vi "AlliGator Decay Graph Panel.vi"() -> ()   [LabVIEW 2021, in "AlliGator Decay Graph.lvlib"]
uses:
  AlliGator Decay Graph.lvlib
  AlliGator Decay Graph Ctrl Refnums.ctl
  Globals, Variables, Constants/AlliGator Refnums List.ctl
  Settings/AlliGator Settings List.ctl
  Graphs/XY Graph/XY Graph Event.ctl
  <vilib>/Utility/miscctls.llb/LVPoint32TypeDef.ctl
  Action Engine/AlliGator Q Element.ctl
  Action Engine/AlliGator Q Event.ctl
  Variant/Variant to Data/Variant to Boolean.vi
  Settings/AlliGator Settings+.lvlib
  Variant/Variant to Data/Variant to Data.lvlib
  Notebook/Notebook.lvlib
  Action Engine/AlliGator Action Engine.lvlib
  GUI/GUI.lvlib
  GUI/AlliGator GUI.lvlib
  Error/Error.lvlib
  Graphs/XY Graph/XY Graph Add-Ons.lvlib
  Python Plugins API/AlliGator Python Plugins.lvlib
  Decay Analysis/Decay Processing/AlliGator Decay Processing.lvlib
  Utilities/Utilities.lvlib
panel:
  out "Decay Integrated Intensity":dbl=46949635.0 caption="Bkgd-subtracted Intensity" format="%#_5g"
  out "Decay Background":dbl caption="Background" format="%#_5g"
  out "Decay Lifetime":dbl[unit] caption="Lifetime" format="%#_5g"
  in  "Decay Graph Active":bool=TRUE
  in  "Pin Button":bool=TRUE
  out "Decay Graph TipStrip":string caption="Lifetime Graph TipStrip"
  out "Decay Graph":cluster{"X Array":dbl[], "Y Array":dbl[]}[](graph)
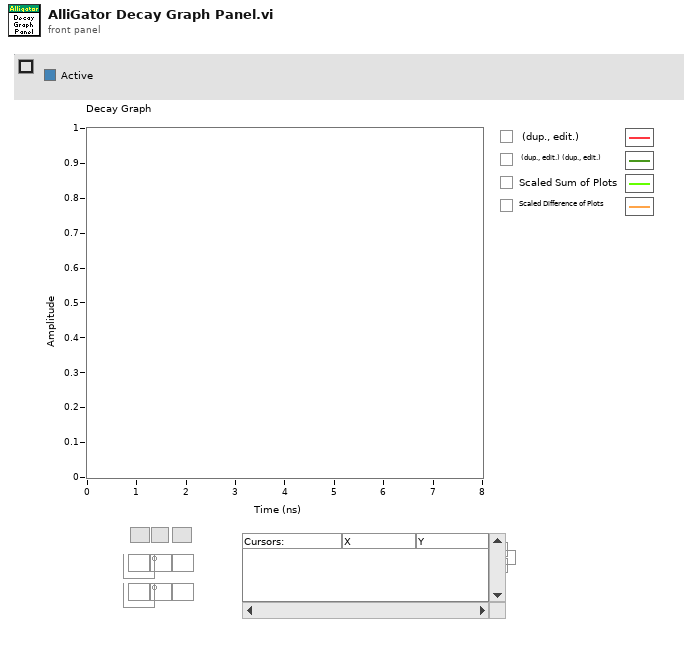
[diagram p1: front panel]
types:
  T1 = typedef "AlliGator GUI.lvlib/AlliGator Refnums List.ctl" = enum16{"---------- AlliGator Control Refnums ----------", "AlliGator Tab Control Refnum", "Dataset Ctrl Refnums", "Image Histogram Ctrl Refnums", "Intensity Time Trace Ctrl Refnums", "Decay Graph Ctrl Refnums", "Decay Statistics Graph Ctrl Refnums", "Phasor Graph Ctrl Refnums", "Phasor Ratio Graph Ctrl Refnums", "Phasor Plot Ctrl Refnums", "Lifetime & Other Parameters Ctrl Refnums", "Decay Fit Parameter Map Ctrl Refnums", "Parameter Map Ctrl Refnums", "Other AlliGator Ctrl Refnums", "---------- AlliGator Menu Refnums ----------", "AlliGator Menu", "---------- IO Device ID ----------", "Mouse ID", "Keyboard ID"}
  T2 = typedef "AlliGator Decay Graph.lvlib/AlliGator Decay Graph Ctrl Refnums.ctl" = cluster{"Decay Graph":refnum<vi>, "Decay Graph Active":refnum<vi>, "Decay Background":refnum<vi>, "Decay Integrated Intensity":refnum<vi>, "Decay Lifetime":refnum<vi>}
  T3 = cluster{"Event Registration Refnum":refnum<event-registration>, "Event Registration Refnum":refnum<event-registration>}
  T4 = typedef "AlliGator Settings+.lvlib/AlliGator Settings List.ctl" = enum16{"GUI:Visible Settings Tab", "GUI:Last Run Version", "Source Image:Use Image Histogram for Contrast", "Source Image:Low Count Pixels Rejection Options", "Source Image:High Count Pixels Rejection Options", "Source Image:Use Image Brightness", "Source Image:Blend Overlay with Image Background", "Source Image:Use Fixed ROI Diameter", "Source Image:ROI Diameter", "Source Image:ROI Center Color", "Source Image:Peak Threshold", "Source Image:Intensity Threshold", "Source Image:Image Binning Options", "Source Image:Image Smoothing Options", "Source Image:Image Histogram Active", "Source Image:Invert Binary Mask", "Source Image:Hot Pixel Removal", "Source Image:Overlay Analyzed ROI Center", "Source Image:Auto-Adjust Contrast", "Source Image:Histogram Lower Percentile", "Source Image:Histogram Upper Percentile", "Source Image:Lock ROI with Maps", "Source Image:Save Source Image", "Source Image:Scale Bar Options", "Source Image:Image Resolution (Pixel Size)", "Source Image:Flatfield Correction", "Source Image:Show Dead Left Columns Correction", "Source Image:Dead Left Columns Correction", "Source Image:Image Pre-Processing Operations Order", "Source Image:Overlay ROI Median", "Source Image:Median Overlay Color", "Data Information:Gate Width", "Data Information:Nanotime Gate Separation", "Data Information:Macrotime Gate Separation", "Data Information:Gate Step", "Data Information:# Gates", "Data Information:Gate Image Exposure", "Data Information:Gate Image Integration", "Data Information:Gates to Skip", "Data Information:Gates to Keep", "Data Information:Define Gates to", "Data Information:Channel Name", "Data Information:Available Channel Names", "Data Information:Channel Arithmetic", "Data Information:Background File Subtraction", "Data Information:Background File", "Data Information:Background Scaling Factor", "Data Information:Background Pile-up Correction", "Data Information:Background Pixel Well Capacity", "Data Information:Laser Period", "Data Information:SYNC Period", "Data Information:Pile-up Correction", "Data Information:Pixel Well Capacity", "Data Information:Dataset Scaling Factor", "Fluorescence Decay_Decay Pre-Processing:Reverse Gates", "Fluorescence Decay_Decay Pre-Processing:Verbose Decay Pre-Processing", "Fluorescence Decay_Decay Pre-Processing:Use Decay Pre-Processing", "Fluorescence Decay_Decay Pre-Processing:Background Subtraction", "Fluorescence Decay_Decay Pre-Processing:Background Definition Range", "Fluorescence Decay_Decay Pre-Processing:Baseline Subtraction Method", "Fluorescence Decay_Decay Pre-Processing:Decay Pre-Processing Operations Order", "Fluorescence Decay_Decay Pre-Processing:Smoothing Parameter", "Fluorescence Decay_Decay Pre-Processing:Shift Decay", "Fluorescence Decay_Decay Pre-Processing:Decay Shift Parameters", "Fluorescence Decay_Decay Pre-Processing:Fold Decay", "Fluorescence Decay_Decay Pre-Processing:# Folds", "Fluorescence Decay_Decay Pre-Processing:1-Normalize Decay", "Fluorescence Decay_Decay Pre-Processing:[0-1]-Normalize Decay", "Fluorescence Decay_Decay Pre-Processing:Smoothen Decay", "Fluorescence Decay_Decay Pre-Processing:Extrapolate Decay", "Fluorescence Decay_Decay Pre-Processing:Use Periodicity", "Fluorescence Decay_Decay Pre-Processing:Use Cursors", "Fluorescence Decay_Decay Pre-Processing:Tail Fraction", "Fluorescence Decay_Decay Pre-Processing:Head Fraction", "Fluorescence Decay_Decay Pre-Processing:Additional Points", "Fluorescence Decay_Decay Pre-Processing:Straighten Decay", "Fluorescence Decay_Decay Pre-Processing:Constant Background", "Fluorescence Decay_Decay Pre-Processing:Pixel-Normalize Decay", "Fluorescence Decay_Advanced Analysis:Extract IRF instead of Decay", "Fluorescence Decay_Advanced Analysis:IRF Extraction Options", "Fluorescence Decay_Advanced Analysis:IRF Optimization Options", "Fluorescence Decay_Advanced Analysis:Square Pulse Options", "Fluorescence Decay_Advanced Analysis:IRF Order", "Fluorescence Decay_Advanced Analysis:IRF Time Constants", "Fluorescence Decay_Advanced Analysis:Wavelet Analysis Options", "Fluorescence Decay_Advanced Analysis:Average Lifetime Options", "Fluorescence Decay_Fit Options:Fit Options", "Fluorescence Decay_Fit Options:Use Legacy Fitting Approach", "Fluorescence Decay_Fit Options:Use Data Information Laser Period", "Fluorescence Decay_Fit Parameters:Displayed Fit Parameters", "Fluorescence Decay_Fit Parameters:Fit Parameter Constraints", "Fluorescence Decay_Fit Parameters:Export Tabulated Results", "Fluorescence Decay_Fit Parameters:MLE Baseline Offset Type", "Fluorescence Decay_Fit Parameters:MLE Baseline Offset", "Fluorescence Decay_Fit Parameters:Guess Parameter Names", "Fluorescence Decay_Fit Parameters:Guess Parameter Values", "Fluorescence Decay_Fit Parameters:Guess Parameters Options", "Fluorescence Decay_Fit Parameters:Optimal Offset Selection Criterion", "Fluorescence Decay_Styles:Show Last Decay Only", "Fluorescence Decay_Styles:Decay Graph Color Array", "Fluorescence Decay:Decay Graph Active", "Fluorescence Decay Statistics:Min Peak Value", "Fluorescence Decay Statistics:Reject Low Decay Peak Pixels", "Fluorescence Decay Statistics:Reject High Decay Peak Pixels", "Fluorescence Decay Statistics:Max Peak Value", "Time Traces:Use File Timestamp", "Time Traces:Time Step", "Time Traces:Use Intensity Correction File", "Time Traces:Intensity Correction File", "Phasor Plot:Phasor Plot Smoothing Options", "Phasor Plot:Phasor Plot Size", "Phasor Plot:Phasor Plot Graphics Options", "Phasor Plot:Cumulative Phasor Plot", "Phasor Plot:Use Phasor Brightness", "Phasor Plot:Blend Overlay with Phasor Background", "Phasor Plot:Save Phasor Plot", "Phasor Plot:Show References", "Phasor Plot:Phasor Ratio Decay Range", "Phasor Plot:Exponential Fading", "Phasor Plot:Phasor Ratio Reference Colors", "Phasor Plot:Reference Radius", "Phasor Plot:Show Color Map Vertices", "Phasor Plot:Phasor Plot Active", "Phasor Plot:Phasor Ratio Color Map Type", "Phasor Plot:Phasor Ratio Color Map", "Phasor Plot:Phasor Ratio Display Range", "Phasor Plot:Selected Image ROI(s)", "Phasor Plot:All Image ROIs", "Phasor Plot:Selected Phasor Plot ROI(s)", "Phasor Plot:All Phasor Plot ROIs", "Phasor Plot:Phasor Ratio Color-Coded Quantity", "Phasor Plot:Store Phasor Harmonics", "Phasor Plot:Draw Reference Segment", "Phasor Plot:User-Defined Quantity", "Phasor Plot:Color Scale High Color", "Phasor Plot:Color Scale Low Color", "Phasor Plot:Intensity-weighted Phasor Plot", "Phasor Graph:Phasor Frequency", "Phasor Graph:Phasor Ratio Type", "Phasor Graph:Pixel-level Phasor Computation", "Phasor Graph:Save Phasor Graph", "Phasor Graph:Phasor Graph Active", "Phasor Graph:Phasor SDV Options", "Phasor Graph:Intensity-weighted Phasor Graph", "Phasor Graph:Define Shortest Lifetime as", "Phasor Calibration:Use Backup Calibration if needed", "Phasor Calibration:Backup Calibration Type", "Phasor Calibration:Calibration Type", "Phasor Calibration:Calibration Lifetime", "Phasor Calibration:Calibration Map Algorithm", "Single-Exponential Phasor Locus (SEPL):Gate Parameters", "Single-Exponential Phasor Locus (SEPL):User-defined Gate", "Single-Exponential Phasor Locus (SEPL):User-defined IRF", "Single-Exponential Phasor Locus (SEPL):Phasor Parameters", "Single-Exponential Phasor Locus (SEPL):Decay & IRF Parameters", "Single-Exponential Phasor Locus (SEPL):Display Parameters", "Lifetime Analysis:Decay Analysis Parameters", "Lifetime Analysis:Lifetime Map Active", "Plugins:Python Settings", "Miscellaneous:Verbose Mode", "Miscellaneous:Beep after Script", "Miscellaneous:Saved Image File Format", "Miscellaneous:Exported Gate Image Settings", "Miscellaneous:Include Loading in Timing", "Miscellaneous:Verbose Settings Mode", "Miscellaneous:Histogram Options", "Miscellaneous:Beep on Error", "Miscellaneous:# Logical Processors Used", "Miscellaneous:ROI Description Max Characters", "Miscellaneous:Verbose Error Mode", "Miscellaneous:Transparent Mask Color"}
  T5 = typedef "XY Graph Add-Ons.lvlib/XY Graph Event.ctl" = cluster{"Item Tag":string, "XY Graph Refnum":refnum<vi>, "Coords":T6, "Item Path":string}
  T6 = typedef "LVPoint32TypeDef.ctl" = cluster{"Horizontal":i32, "Vertical":i32}
  T7 = enum16{"0", "1", "2", "3", "4", "5", "6", "7", "8", "9", "A", "B", "C", "D", "E", "F", "G", "H", "I", "J", "K", "L", "M", "N", "O", "P", "Q", "R", "S", "T", "U", "V", "W", "X", "Y", "Z", "F1", "F2", "F3", "F4", "F5", "F6", "F7", "F8", "F9", "F10", "F11", "F12", "F13", "F14", "F15", "ADD", "BACK", "BACKSLASH", "CAPITAL", "COMMA", "DECIMAL", "DELETE", "DIVIDE", "DOWN", "END", "EQUALS", "ESCAPE", "GRAVE (`)", "HOME", "INSERT", "LBRACKET", "LCONTROL", "LEFT", "L ALT", "LSHIFT", "LWIN", "MINUS", "MULTIPLY", "NEXT", "NUMLOCK", "NUMPAD_0", "NUMPAD_1", "NUMPAD_2", "NUMPAD_3", "NUMPAD_4", "NUMPAD_5", "NUMPAD_6", "NUMPAD_7", "NUMPAD_8", "NUMPAD_9", "PAUSE", "PERIOD", "PRIOR (PG UP)", "RBRACKET", "RCONTROL", "RETURN", "RIGHT", "R ALT", "RSHIFT", "RWIN", "SCROLL", "SEMICOLON", "SLASH", "SPACE", "SUBTRACT", "TAB", "UP", "ENTER (num pad)", "' (quote)"}
  T8 = typedef "AlliGator Action Engine.lvlib/AlliGator Q Element.ctl" = cluster{"AlliGator Q Event":T9, "Data":variant}
  T9 = typedef "AlliGator Action Engine.lvlib/AlliGator Q Event.ctl" = enum16{"---- Files ----", "Files:Set Batch Export Files To Save", "Files:Set Dataset Loading & Pre-processing Options", "Files:Check #Frames in Dataset", "Files:Increment Frame Index", "Files:Open Mask Image", "Files:Open White Light Image", "Files:Open Single Dataset", "Files:New Folder of Folders Selected", "Files:Load File (all Types)_Scriptable", "Files:Move Flattened Series to Folders Series", "Files:Select Folder", "Files:Load FLI Dataset", "Files:Load Swiss SPAD 1 Dataset", "Files:Load Swiss SPAD 2 Dataset", "Files:Load .sdt FLI Dataset", "Files:Load .ptu FLI Dataset", "Files:Load .bin FLI Dataset", "Files:Load Single Gate Image Folder", "Files:Load I/m/phi Dataset (deprecated)", "Files:Load Single Image", "Files:Subtract Background File", "Files:Export FLI Dataset", "Files:Load HDF5 FLI Dataset", "Files:Set Destination File Path", "Files:Save Mask Image", "Files:Batch Conversion", "Files:New Folder Selected", "Files:Close FLI Dataset", "Files:Close FLI Dataset Series", "Files:Close White Light Image", "Files:Close Mask Image", "---- FLI Dataset ----", "FLI Dataset:Channel Arithmetic", "FLI Dataset:Export Average Lifetime Map as ASCII", "FLI Dataset:Export User-Defined Quantity Map as ASCII", "FLI Dataset:Python Function FLI Dataset Event", "FLI Dataset:ROI Analysis", "FLI Dataset:Tilted Logistic Square Gated IRF Characteristics Map", "FLI Dataset:Logistic Square Gated IRF Characteristics Map", "FLI Dataset:Square Gated IRF Characteristics Map", "FLI Dataset:Multi-ROI Single-Pixel Phasor Analysis", "FLI Dataset:Multi-ROI Single-Pixel NLSF Analysis", "FLI Dataset:All ROIs IRF Extraction", "FLI Dataset:All ROIs Decay Fit Non-Interactive (Fast + Individual IRF)", "FLI Dataset:All ROIs Phasor Analysis", "FLI Dataset:All ROIs Decay Fit", "FLI Dataset:Fluorescence Decay Statistics", "FLI Dataset:Update Decay Statistics Graph", "FLI Dataset:Get Decay from ROI", "FLI Dataset:All ROIs Average Lifetimes", "FLI Dataset:Save/Load Local IRFs", "FLI Dataset:Clear Local IRFs", "FLI Dataset:Phasor Calibration Maps (# Gates Series) Script", "FLI Dataset:Calibrated Phasor Map Series", "---- FLI Dataset Series ----", "FLI Dataset Series:Sum All Datasets in Series", "FLI Dataset Series:Add Dataset to Accumulated Dataset", "FLI Dataset Series:Display Accumulated Dataset", "FLI Dataset Series:Clear Dataset Series Sum", "FLI Dataset Series:Time-Series Analysis (NLSF)", "FLI Dataset Series:Time-Series Analysis (Phasor)", "---- Image ----", "Image:Update Image Profile Plots", "Image:Image Histogram Cursor Move", "Image:Image Histogram", "Image:Image Contrast", "Image:Set Image Histogram Cursor Move Flag", "Image:Clear Image Overlay", "Image:Use ROI as Search Area", "Image:Set ROI Diameter", "Image:Save Image Data as TIFF", "Image:Save Displayed Image with Overlay", "Image:Save Image Overlay Only", "Image:Save Image as Hot Pixel Mask", "Image:Change Source Image Color Palette", "Image:Copy Image to Clipboard", "Image:Source Image ROI Selection", "Image:Delete All ROIs", "Image:Delete All Unselected ROIs", "Image:Delete ROI", "Image:Merge All ROIs", "Image:Store ROI", "Image:Source Image ROI Storage", "Image:Export ROI Description to Notebook", "Image:Save ROI", "Image:Load ROI", "Image:Paste ROI Definition", "Image:Clear ROI", "Image:Identify ROIs in Mask Image", "Image:Create Complementary ROI", "Image:Create Contour ROI", "Image:Create ROI(s) from Pixels with Peak above Min_Scriptable", "Image:Create ROI(s) from Pixels with Intensity above Min_Scriptable", "Image:Compute ROI Statistics", "Image:Delete ROI(s) based on ROI Characteristics", "Image:Create ROI Grid", "Image:ROI to Individual Pixel ROIs", "Image:Python Function Source Image Event", "Image:Show Phasor Calibration Map ROI Centers", "Image:Convert ROI to Mask Image", "Image:Mouse Move", "Image:Mouse Up", "Image:Set Source Image Mouse Move Flag", "Image:Add Scale Bar Overlay", "Image:Delete Existing ROIs Option", "Image:Overlay ROI Median", "Image:Check Current ROI", "Image:Update True Pixel Value", "Image:Use ROI", "---- Decay ----", "Decay:Clear IRF/Reference Plot", "Decay:Add Decay to Graph", "Decay:Smoothen Plot", "Decay:Smoothen Plot Tail", "Decay:Average Selected Plots", "Decay:Extract IRF", "Decay:Optimal IRF Extraction", "Decay:Threshold IRF", "Decay:Fit to Model IRF", "Decay:Fit IRF to Square Gate", "Decay:Fit IRF to Logistic Square Gate", "Decay:Fit IRF to Tilted Logistic Square Gate", "Decay:Create Bounding Cursors Set", "Decay:Export Bounding Cursors Definition to Notebook", "Decay:Denoise Plot", "Decay:Compute Cumulative Function", "Decay:Use as Reference Decay", "Decay:Show Reference Decay/IRF", "Decay:Extrapolate Decay", "Decay:Create Head & Tail Bounding Cursors", "Decay:Store Cursor-defined Head & Tail Fractions", "Decay:Rebin Plot", "Decay:1-Normalize Decay", "Decay:[0-1]-Normalize Plot", "Decay:Straighten Decay", "Decay:Shift Decay", "Decay:Fold Decay", "Decay:Fit Decay", "Decay:Global Fit of Selected Decays", "Decay:Post Global Fit Script", "Decay:Add Global Fit Parameters to Graph", "Decay:Add Decay Parameter(s) to Plot (Graph)", "Decay:Export Decay to Phasor Graph", "Decay:Compute Average Lifetime", "Decay:Plot Convolution", "Decay:Graph Tip Strip Update", "---- Decay Statistics ----", "Decay Statistics:Tip Strip Update", "---- Intensity Time Trace ----", "Intensity Time Trace:Use File Timestamp", "Intensity Time Trace:Load Intensity Corrections File", "Intensity Time Trace:Clear Intensity Corrections File", "Intensity Time Trace:Tip Strip Update", "---- Phasor Plot ----", "Phasor Plot:Build Phasor Plot", "Phasor Plot:Change Phasor Plot Color Palette", "Phasor Plot:Adjust Phasor Plot Display Range", "Phasor Plot:Highlight Image ROI in Phasor Plot", "Phasor Plot:Save Phasor Plot Image with Overlay", "Phasor Plot:Export Complex Phasor Map", "Phasor Plot:Export Phasor Ratio Map", "Phasor Plot:Export Average Lifetime Map", "Phasor Plot:Compute Phase Lifetime Histogram", "Phasor Plot:Compute Phasor Ratio Histogram", "Phasor Plot:Compute Phase Lifetime vs Intensity Scatter Plot", "Phasor Plot:Weber 2-Component Decomposition", "Phasor Plot:Update Phasor Color Map Vertices", "Phasor Plot:Clear Phasor Overlay", "Phasor Plot:Use Segment Extremities as References", "Phasor Plot:Use UC/Segment Intersections as References", "Phasor Plot:Use UC/Principal Axis Intersections as References", "Phasor Plot:Use UC/Linear Fit Intersections as References", "Phasor Plot:Update Phasor Plot Reference", "Phasor Plot:Show Local Phasor Info in Phasor Plot", "Phasor Plot:Update Phasor Plot State", "Phasor Plot:Phasor Plot ROI Storage", "Phasor Plot:Phasor Plot ROI Selection", "Phasor Plot:Python Function Phasor Plot Event", "Phasor Plot:Overlay Phasor ROI, Ratio or Map in Source Image", "Phasor Plot:Compute Decay of Selected Phasors", "Phasor Plot:Phasor at Image Pixel", "Phasor Plot:Mouse Move", "Phasor Plot:Mouse Up", "Phasor Plot:Display Range Mouse Move", "Phasor Plot:Set Mouse Move Flag", "Phasor Plot:Update True Phasor Plot Value", "---- Phasor Graph ----", "Phasor Graph:Get Phasor Value", "Phasor Graph:Create New Phasor Plot Dialog", "Phasor Graph:Update Last Phasor Value", "Phasor Graph:Update Phasor (m, phi)", "Phasor Graph:Remove Single Phasor from Plot", "Phasor Graph:Add Single Phasor to Plot", "Phasor Graph:Remove Phasor Plot", "Phasor Graph:Remove Selected Phasor Plots", "Phasor Graph:Clear Phasor Data", "Phasor Graph:Clear Phasor Graph", "Phasor Graph:Cursor Move", "Phasor Graph:Draw Cursor Connecting Line", "Phasor Graph:Clear Cursor Connecting Line", "Phasor Graph:Find UC Intersection", "Phasor Graph:Use UC/Cursor-Defined Line Intersections", "Phasor Graph:Use Selected Plots Fitted Line/UC Intersections", "Phasor Graph:Use Selected Plots Principal Axis/UC Intersections", "Phasor Graph:Show Single Phasor", "Phasor Graph:Save Single Phasor Plot", "Phasor Graph:Save All Phasor Plots", "Phasor Graph:Load Phasor Plot(s)", "Phasor Graph:Phasor Multiplication", "Phasor Graph:Compute Average Phasor", "Phasor Graph:Compute Multiple Average Phasors (Selected Plots)", "Phasor Graph:Export Single Phasor Plot Phase Lifetimes", "Phasor Graph:Parameter 2 vs Parameter 1 Scatter Plot", "Phasor Graph:Use Cursor n Location", "Phasor Graph:Set Reference n to Current Phase Lifetime Value", "Phasor Graph:Set Reference n to Lifetime Value", "Phasor Graph:Set Cursor n Location", "Phasor Graph:Save Phasor Graph Image", "Phasor Graph:Update SEPL Plot", "Phasor Graph:Export Single Phasor Plot Data", "Phasor Graph:Export Selected Phasor Plots Data", "Phasor Graph:Python Function Phasor Graph Event", "Phasor Graph:Tip Strip Update", "---- Calibration ----", "Calibration:Set Calibration Type", "Calibration:Load/Save Phasor Calibration", "Calibration:Load/Save Phasor Calibration Series", "Calibration:Load/Save Phasor Calibration Map", "Calibration:Use as Calibration", "Calibration:Compute Optimal Calibration from Phasor References", "Calibration:Clear Phasor Calibration", "Calibration:Single Phasor Calibration Information", "Calibration:Use as Calibration Series", "Calibration:Use as Calibration Map", "Calibration:Clear Calibration Series", "Calibration:Phasor Calibration Series Information", "Calibration:Clear Calibration Map", "Calibration:Phasor Calibration Map Information", "Calibration:Apply Phasor Calibration", "Calibration:Update Single Plot Calibration", "Calibration:Update Multiple Plots Calibration", "Calibration:Clear Single Plot Calibration", "Calibration:Clear All Plots Calibrations", "Calibration:Clear Plot(s) Calibration(s)?", "---- Phasor Ratio ----", "Phasor Ratio:Clear Reference n", "Phasor Ratio:Toggle Selected Plot(s)  Lock to Reference 1", "Phasor Ratio:Use as Reference n", "Phasor Ratio:Send Reference n to Notebook", "Phasor Ratio:Toggle Selected Plot(s)  Lock to Reference 2", "Phasor Ratio:Compute Phasor Ratio at Mouse Location", "Phasor Ratio:Compute Phasor Plot's Average Phasor Ratio", "Phasor Ratio:Compute Time-Series Phasor Ratios", "Phasor Ratio:Fit Line to Phasor Ratio Plot", "Phasor Ratio:Save References", "Phasor Ratio:Load References", "Phasor Ratio:Update Phasor Reference 1", "Phasor Ratio:Update Phasor Reference 2", "Phasor Ratio:Move Cursor n to Reference n", "Phasor Ratio:Use as Phasor Reference 1 Lifetime", "Phasor Ratio:Use as Phasor Reference 2 Lifetime", "Phasor Ratio:Export Phasor Ratio Map as ASCII", "Phasor Ratio:Tip Strip Update", "---- Lifetime & Other Parameters Graph ----", "Lifetime:Compute Sliced Mean, SDV and CV Plots", "Lifetime:Plot Decay Shifts", "Lifetime:Plot Histogram", "---- Decay Fit Parameter Map ----", "Decay Fit Parameter Map:Export ROI NLSF Data as ASCII", "Decay Fit Parameter Map:Set Decay Fit Parameter Map Selection", "Decay Fit Parameter Map:Build Decay Fit Parameter Map", "Decay Fit Parameter Map:Change Decay Fit Parameter Map Color Palette", "Decay Fit Parameter Map:Export Decay Fit Parameter Map Data as ASCII", "Decay Fit Parameter Map:Export All Decay Fit Parameter Maps Data as ASCII", "Decay Fit Parameter Map:Selected Parameter Scatterplot", "Decay Fit Parameter Map:Parameter 2 vs Parameter 1 Scatterplot", "Decay Fit Parameter Map:Save Decay Fit Parameter Map Image", "Decay Fit Parameter Map:Save-Load IRFs & Fit Data", "Decay Fit Parameter Map:Update Local Decay Plots", "Decay Fit Parameter Map:Python Function Decay Fit Parameters Map Event", "Decay Fit Parameter Map:Overlay Decay Fit Parameter Map in Source Image", "Decay Fit Parameter Map:Selected Parameter vs Intensity Scatterplot", "Decay Fit Parameter Map:Mouse Up", "Decay Fit Parameter Map:Mouse Move", "Decay Fit Parameter Map:Display Range Mouse Move", "Decay Fit Parameter Map:Change Map Resolution", "Decay Fit Parameter Map:Variance Significance Maps", "Decay Fit Parameter Map:Fit Result Constraints Window", "Decay Fit Parameter Map:Use ROI", "---- Parameter Map ----", "Parameter Map:Export ROI Parameters Data as ASCII", "Parameter Map:Add Parameter Map Set", "Parameter Map:Delete Parameter Map Set", "Parameter Map:Update Parameter List", "Parameter Map:Build Parameter Map", "Parameter Map:Change Parameter Map Color Palette", "Parameter Map:Export Parameter Map Data as ASCII", "Parameter Map:Export All Parameter Maps Data as ASCII", "Parameter Map:Selected Parameter Scatterplot", "Parameter Map:Parameter 2 vs Parameter 1 Scatterplot", "Parameter Map:Selected Parameter vs Intensity Scatterplot", "Parameter Map:Save Parameter Map Image", "Parameter Map:Save-Load IRFs & Parameter Maps (TODO)", "Parameter Map:Set Parameter Map Selection", "Parameter Map:Python Function Parameter Map Event", "Parameter Map:Overlay Parameter Map in Source Image", "Parameter Map:Update Local Decay Plots", "Parameter Map:Mouse Up", "Parameter Map:Mouse Move", "Parameter Map:Display Range Mouse Move", "Parameter Map:Use ROI", "---- Generic Graph ----", "Generic Graph:Generic XY Graph Event", "Generic Graph:Python Function XY Graph Event", "Generic Graph:New Plot", "Generic Graph:Save Plot", "Generic Graph:XY Plot Histogram", "Generic Graph:Set XY Graph Plot Name", "Generic Graph:Set Last Cursor Style", "Generic Graph:Tip Strip Update", "---- GUI ----", "GUI:Start Script", "GUI:Type of Displayed Image Changed", "GUI:Gate Image Slide Changed", "GUI:Show Busy Icon", "GUI:Show Busy Icon & Abort Button", "GUI:Hide Busy Icon", "GUI:Hide Busy Icon & Abort Button", "GUI:Abort", "GUI:End Script", "GUI:Start Timing", "GUI:End Timing", "GUI:Set State Indicator", "GUI:Send Parameters JSON Strings to Clipboard", "GUI:Set Gate Step", "GUI:Idle", "GUI:Initialization", "GUI:Quit", "GUI:Increment Dataset Index", "GUI:Set Dataset Index to -1", "GUI:Time Series Slider Moved", "GUI:Time Series Slider Changed", "GUI:Toggle Playback or Loop", "GUI:Playback Script", "GUI:Set Phasor Frequency", "GUI:Open Window", "GUI:Start Test Script", "GUI:End Test Script", "GUI:Set Verbose Mode", "GUI:Set Verbose Settings Mode", "GUI:Initialize Python Session", "DEBUG"}
  T10 = enum16{"0", "1", "2", "3", "4", "5", "6", "7", "8", "9", "A", "B", "C", "D", "E", "F", "G", "H", "I", "J", "K", "L", "M", "N", "O", "P", "Q", "R", "S", "T", "U", "V", "W", "X", "Y", "Z", "F1", "F2", "F3", "F4", "F5", "F6", "F7", "F8", "F9", "F10", "F11", "F12", "F13", "F14", "F15", "ADD", "BACK", "BACKSLASH", "CAPITAL", "COMMA", "DECIMAL", "DELETE", "DIVIDE", "DOWN", "END", "EQUALS", "ESCAPE", "GRAVE (`)", "HOME", "INSERT", "LBRACKET", "LCONTROL", "LEFT", "L ALT", "LSHIFT", "LWIN", "MINUS", "MULTIPLY", "NEXT", "NUMLOCK", "NUMPAD_0", "NUMPAD_1", "NUMPAD_2", "NUMPAD_3", "NUMPAD_4", "NUMPAD_5", "NUMPAD_6", "NUMPAD_7", "NUMPAD_8", "NUMPAD_9", "PAUSE", "PERIOD", "PRIOR (PG UP)", "RBRACKET", "RCONTROL", "RETURN", "RIGHT", "R ALT", "RSHIFT", "RWIN", "SCROLL", "SEMICOLON", "SLASH", "SPACE", "SUBTRACT", "TAB", "UP", "ENTER (num pad)", "' (quote)"}[]
  T11 = typedef "XY Graph Add-Ons.lvlib/XY Graph Refnum.ctl" = refnum<vi>
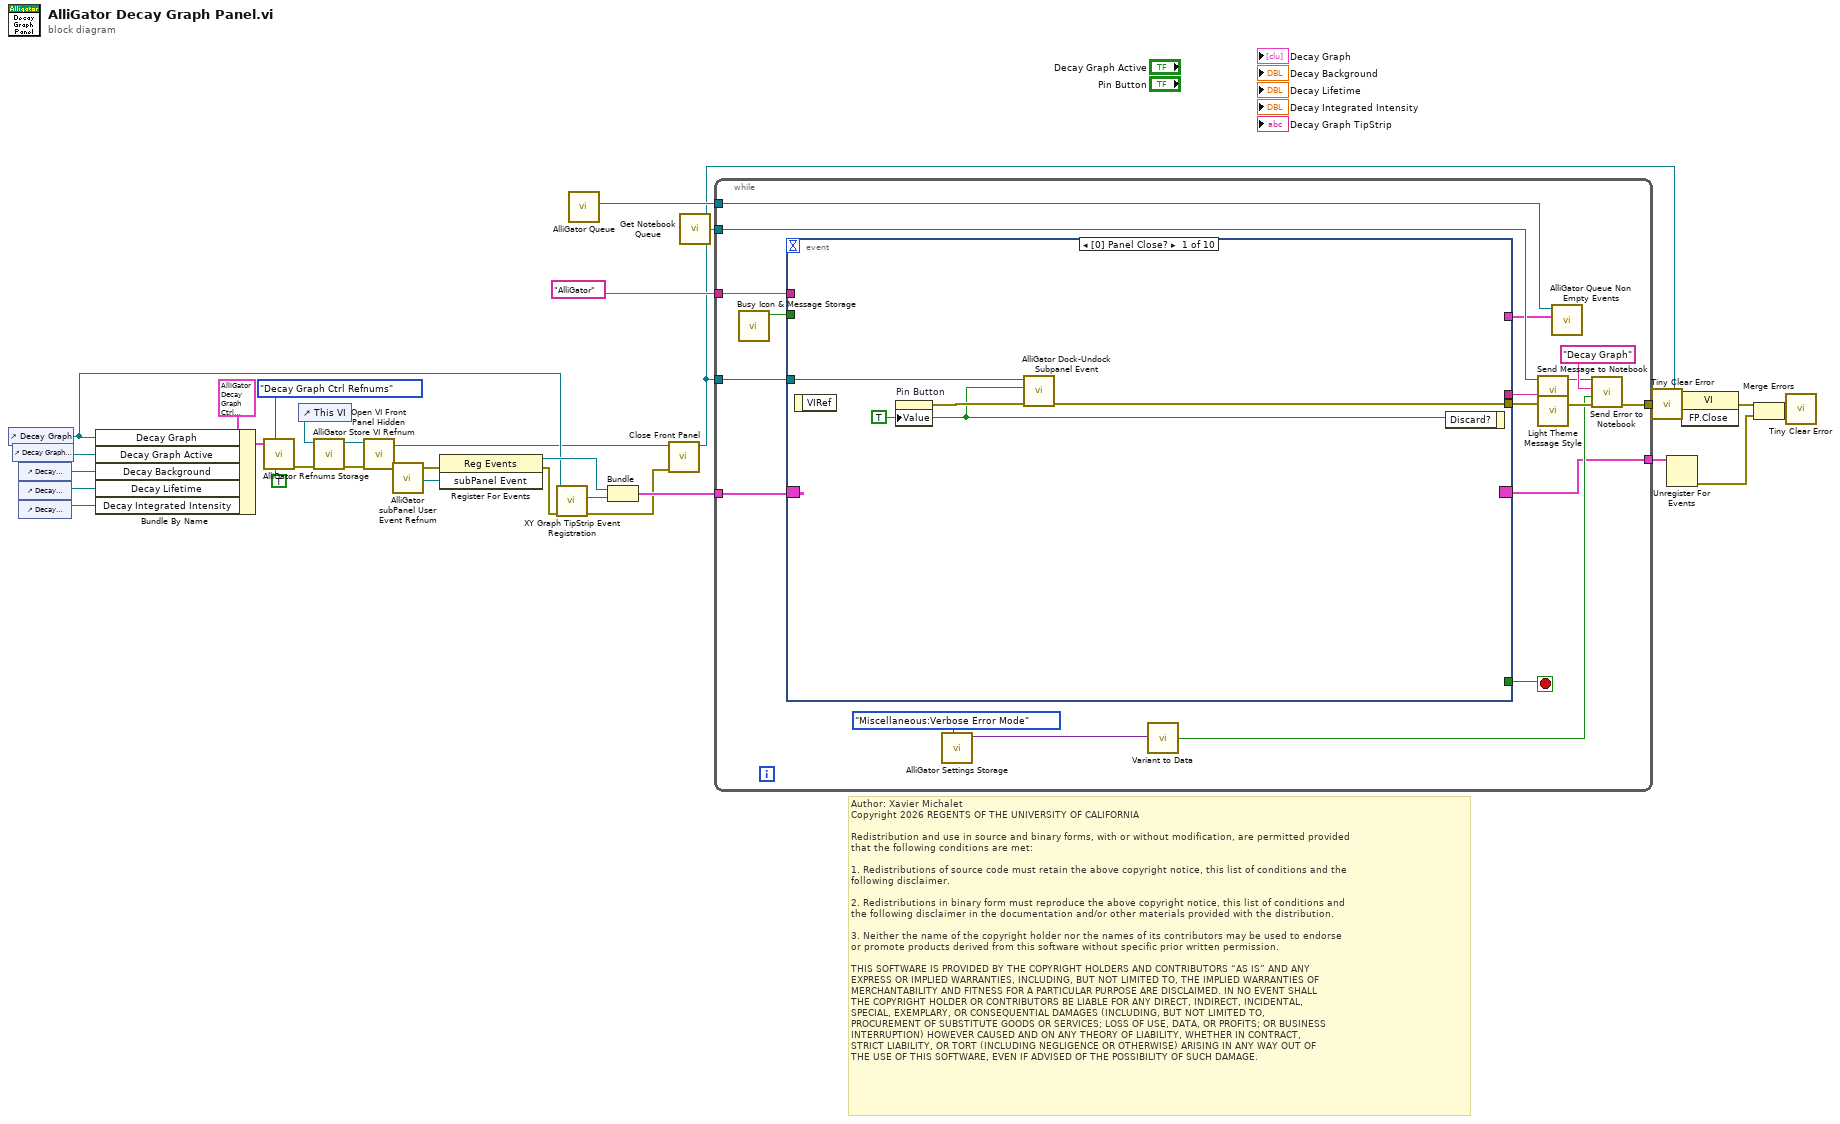
[diagram p0: block diagram]
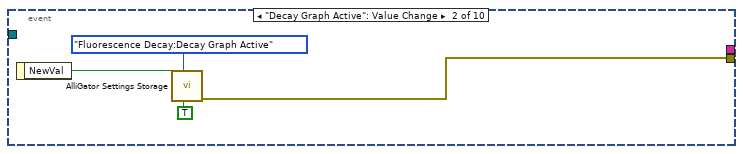
[diagram p2: hidden frame]
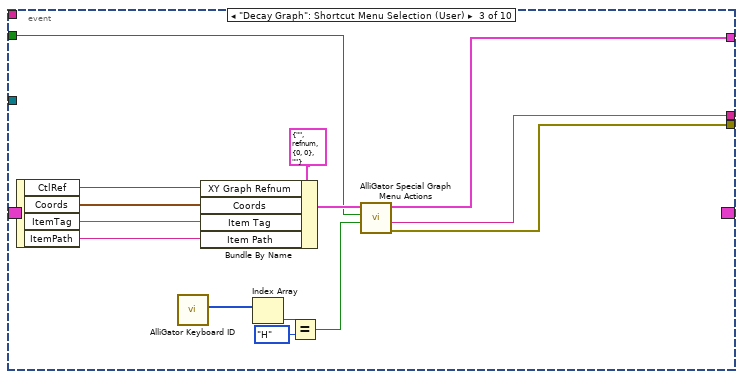
[diagram p3: hidden frame]
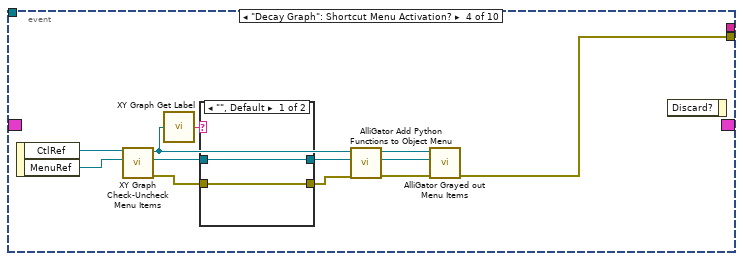
[diagram p4: hidden frame]
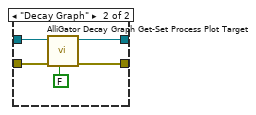
[diagram p5: hidden frame]
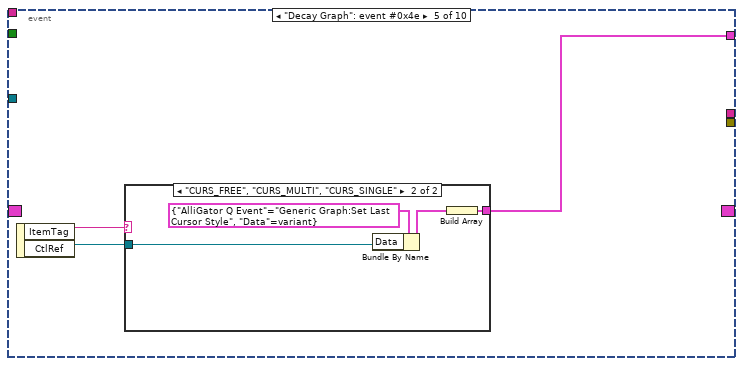
[diagram p6: hidden frame]
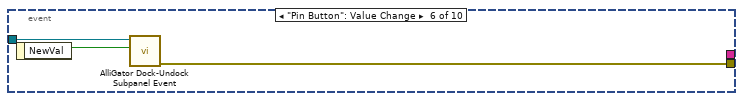
[diagram p8: hidden frame]
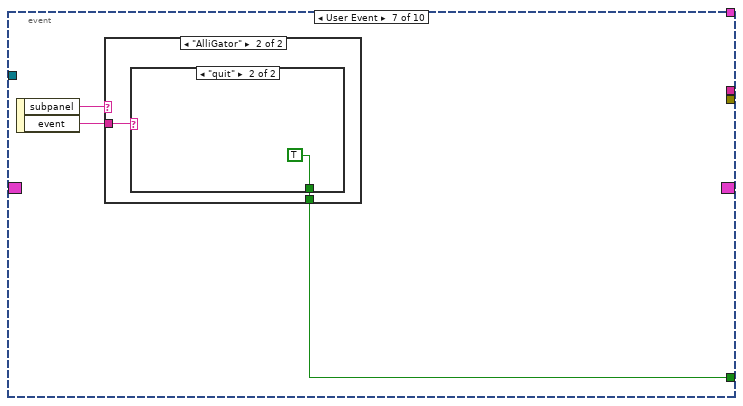
[diagram p9: hidden frame]
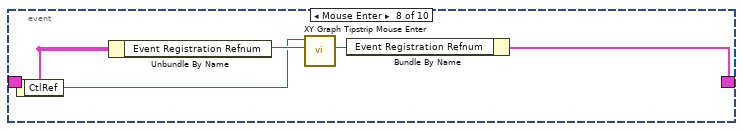
[diagram p12: hidden frame]
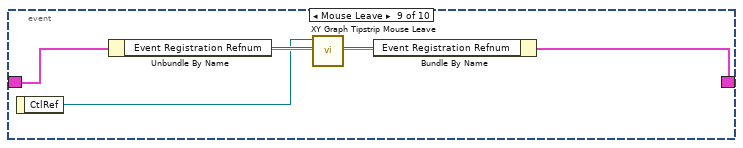
[diagram p13: hidden frame]
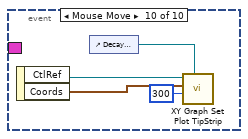
[diagram p14: hidden frame]
diagram:
  # "Author: Xavier Michalet\nCopyright 2026 REGENTS OF THE UNIVERSITY OF CALIFORNIA\n\nRedistribution and use in source and binary forms, with or without modification, are permitted provided\nthat the following conditions are met:\n\n1. Redistributions of source code must retain the above copyright notice, this list of conditions and the\nfollowing disclaimer.\n\n2. Redistributions in binary form must reproduce the above copyright notice, this list of conditions and\nthe following disclaimer in the documentation and/or other materials provided with the distribution.\n\n3. Neither the name of the copyright holder nor the names of its contributors may be used to endorse \nor promote products derived from this software without specific prior written permission.\n\nTHIS SOFTWARE IS PROVIDED BY THE COPYRIGHT HOLDERS AND CONTRIBUTORS “AS IS” AND ANY \nEXPRESS OR IMPLIED WARRANTIES, INCLUDING, BUT NOT LIMITED TO, THE IMPLIED WARRANTIES OF\nMERCHANTABILITY AND FITNESS FOR A PARTICULAR PURPOSE ARE DISCLAIMED. IN NO EVENT SHALL\nTHE COPYRIGHT HOLDER OR CONTRIBUTORS BE LIABLE FOR ANY DIRECT, INDIRECT, INCIDENTAL, \nSPECIAL, EXEMPLARY, OR CONSEQUENTIAL DAMAGES (INCLUDING, BUT NOT LIMITED TO, \nPROCUREMENT OF SUBSTITUTE GOODS OR SERVICES; LOSS OF USE, DATA, OR PROFITS; OR BUSINESS\nINTERRUPTION) HOWEVER CAUSED AND ON ANY THEORY OF LIABILITY, WHETHER IN CONTRACT, \nSTRICT LIABILITY, OR TORT (INCLUDING NEGLIGENCE OR OTHERWISE) ARISING IN ANY WAY OUT OF\nTHE USE OF THIS SOFTWARE, EVEN IF ADVISED OF THE POSSIBILITY OF SUCH DAMAGE."
  n1 = control-ref of="Decay Graph"() -> (w18:refnum<vi>)
  n2 = control-ref of="Decay Graph Active"() -> (w19:refnum<vi>)
  n3 = control-ref of="Decay Background"() -> (w7:refnum<vi>)
  n4 = control-ref of="Decay Lifetime"() -> (w6:refnum<vi>)
  n5 = control-ref of="Decay Integrated Intensity"() -> (w5:refnum<vi>)
  n6 = Bundle By Name(cluster=T2 {"Decay Graph"=refnum, "Decay Graph Active"=refnum, "Decay Background"=refnum, "Decay Integrated Intensity"=refnum, "Decay Lifetime"=refnum} ("Decay Graph Ctrl Refnums"), "Decay Graph"=w18, "Decay Graph Active"=w19, "Decay Background"=w7, "Decay Lifetime"=w6, "Decay Integrated Intensity"=w5) -> (w20:T2)
  n7 = call "AlliGator Refnums Storage.vi"("Get(F)/Set"=TRUE, "AlliGator Refnum List"=AlliGator_Refnums_List."Decay Graph Ctrl Refnums", "Data in"=w20) -> ("Error Out"=w2:errorcluster)  [unwired: 7 in, 1 out]
  n8 = control-ref of="This VI"() -> (w4:refnum<vi>)
  n9 = call "AlliGator Store VI Refnum.vi"("error in (no error)"=w2, "VI Refnum"=w4) -> ("error out"=w1:errorcluster, "VI Refnum (dup)"=w3:refnum<vi>)  [unwired: 7 in, 1 out]
  n10 = call "Open VI Front Panel Hidden.vi"("error in"=w1, "VI in"=w3) -> ("error out"=w12:errorcluster, "VI out"=w11:refnum<vi>)  [unwired: 8 in]
  n11 = call "AlliGator subPanel User Event Refnum.vi"() -> ("subPanel Event"=w28:refnum<user-event>)  [unwired: 9 in]
  n12 = register-events(error in=w12, w28) -> (reference out=w27:refnum<event-registration>, error out=w9:errorcluster)  [unwired: 1 in]
  n13 = call "XY Graph TipStrip Event Registration.vi"("error in (no error)"=w9, "XY Graph Refnum"=w18) -> ("error out"=w8:errorcluster, "Event Registration Refnum"=w16:refnum<event-registration>)  [unwired: 7 in, 1 out]
  n14 = call "AlliGator Queue.vi"() -> ("AlliGator Q"=w30:refnum<queue>)  [unwired: 8 in, 1 out]
  n15 = Bundle("Event Registration Refnum"=w27, "Event Registration Refnum"=w16) -> (w17:T3)  [unwired: 1 in]
  n16 = call "Close Front Panel.vi"("error in (no error)"=w8, "VI in"=w11) -> ("VI out"=w10:refnum<vi>)  [unwired: 8 in, 1 out]
  n17 = call "Get Notebook Queue.vi"() -> ("Notebook Queue"=w31:refnum<queue>)  [unwired: 9 in]
  n18 = while {
    tunnel: w31 -> [w42]
    tunnel: w30 -> [w39]
    tunnel: "AlliGator" ("Sender") -> [w37]
    tunnel: w10 -> [w35]
    tunnel: w17 -> [w34]
    tunnel: [w33] -> w26
    tunnel: [w32] -> w25
    stop <- w49 stop-if-true
    n19 = call "Busy Icon & Message Storage.vi"() -> ("Busy Icon Status (F = busy)"=w36:bool)  [unwired: 9 in, 2 out]
    n20 = event shown="[0] Panel Close?" {
      selector: w34 -> [_ _ _ _ _ _ _ w109 w114 _]
      dyn-events: [_ _ _ _ _ _ _ w107 w112 _] -> w33
      timeout: _ -> [_ _ _ _ _ _ _ _ _ _]
      tunnel: [w52 w54 w58 w72 _ w98 _ _ _ _] -> w43
      tunnel: [_ _ _ _ _ _ w101 _ _ _] -> w49
      tunnel: [_ _ w59 _ _ _ _ _ _ _] -> w40
      tunnel: [_ _ w60 _ w91 _ _ _ _ _] -> w38
      tunnel: w36 -> [_ _ w65 _ _ _ _ _ _ _]
      tunnel: w37 -> [_ _ _ _ _ _ _ _ _ _]
      tunnel: w35 -> [w51 _ _ _ _ w100 _ _ _ _]
      event Panel Close? {
        w50 = TRUE ("Pin Button")
        n21 = event-data() -> ()  [unwired: 1 in, 1 out]
        n22 = property on="Pin Button" class="Bool (strict)"("Value"=w50) -> (error out=w53:errorcluster)  [unwired: 2 in, 1 out]
        n23 = call "AlliGator Dock-Undock Subpanel Event.vi"("Error In"=w53, "Dock?"=w50, "VI in"=w51) -> ("Error Out"=w52:errorcluster)  [unwired: 8 in]
        n24 = event-data("Discard?"=w50) -> ()  [unwired: 1 in, 1 out]
      }
      event "Decay Graph Active": Value Change {
        n25 = event-data() -> ("NewVal"=w56:bool)  [unwired: 1 in]
        n26 = call "AlliGator Settings Storage.vi"("Get(F)/Set"=TRUE, "AlliGator Settings List"=AlliGator_Settings_List."Fluorescence Decay:Decay Graph Active", "Variant Data in"=w56) -> ("Error Out"=w54:errorcluster)  [unwired: 7 in, 1 out]
      }
      event "Decay Graph": Shortcut Menu Selection (User) {
        n27 = event-data() -> ("CtlRef"=w61:refnum<vi>, "Coords"=w64:T6, "ItemTag"=w62:string, "ItemPath"=w63:string)  [unwired: 1 in]
        n28 = call "AlliGator Keyboard ID.vi"() -> ("keys pressed"=w71:T10)  [unwired: 9 in, 2 out]
        n29 = Bundle By Name(cluster=T5 {"Item Tag"="", "XY Graph Refnum"=refnum, "Coords"={"Horizontal"=0, "Vertical"=0}, "Item Path"=""} ("XY Graph Event"), "XY Graph Refnum"=w61, "Coords"=w64, "Item Tag"=w62, "Item Path"=w63) -> (w69:T5)
        n30 = Index Array(array=w71) -> (element=w66:T7)  [unwired: 1 in]
        n31 = Equal?(x=w66, y=T7."H" ("element")) -> (x = y?=w70:bool)
        n32 = call "AlliGator Special Graph Menu Actions.vi"("Help?"=w70, "Animated Busy Icon"=w65, "XY Graph Event"=w69) -> ("Error Out"=w58:errorcluster, "Message"=w59:string, "AlliGator Actions"=w60:T8[])  [unwired: 6 in]
      }
      event "Decay Graph": Shortcut Menu Activation? {
        n33 = event-data() -> ("CtlRef"=w74:refnum<vi>, "MenuRef"=w73:refnum<k9>)  [unwired: 1 in]
        n34 = call "XY Graph Check-Uncheck Menu Items.vi"("Menu in"=w73, "XY Graph Refnum"=w74) -> ("Error Out (dup)"=w83:errorcluster, "Menu out"=w78:refnum<k9>, "XY Graph Refnum dup"=w76:T11)  [unwired: 6 in, 1 out]
        n35 = call "XY Graph Get Label.vi"("XYGraph"=w76) -> ("Graph Label"=w75:string)  [unwired: 8 in]
        n36 = case shown="\"\", Default" w75 {
          tunnel: w83 -> [w84 w90]
          tunnel: [w84 w89] -> w79
          tunnel: w78 -> [w85 w88]
          tunnel: [w85 w87] -> w77
          frame "", Default {
          }
          frame "Decay Graph" {
            n37 = call "AlliGator Decay Graph Get-Set Process Plot Target.vi"("Get (F)/Set"=FALSE, "Error In"=w90, "Menu"=w88) -> ("Error Out (dup)"=w89:errorcluster, "Menu"=w87:refnum<k9>)  [unwired: 6 in, 1 out]
          }
        }
        n38 = call "AlliGator Add Python Functions to Object Menu.vi"("error in (no error)"=w79, "Menu in"=w77, "Object Refnum"=w76) -> ("error out"=w82:errorcluster, "Menu out"=w81:refnum<k9>, "Object Refnum dup"=w80:refnum<vi>)  [unwired: 6 in]
        n39 = call "AlliGator Grayed out Menu Items.vi"("error in (no error)"=w82, "Menu in"=w81, "Object Refnum"=w80) -> ("error out"=w72:errorcluster)  [unwired: 7 in, 1 out]
        n40 = event-data() -> ()  [unwired: 2 in, 1 out]
      }
      event "Decay Graph": event #0x4e {
        n41 = event-data() -> ("ItemTag"=w92:string, "CtlRef"=w93:refnum<vi>)  [unwired: 1 in]
        n42 = case shown="\"CURS_FREE\", \"CURS_MULTI\", \"CURS_SINGLE\"" w92 {
          tunnel: w93 -> [_ w94]
          tunnel: [_ w96] -> w91
          frame "", Default {
          }
          frame "CURS_FREE", "CURS_MULTI", "CURS_SINGLE" {
            n43 = Bundle By Name(cluster=T8 {"AlliGator Q Event"=enum."Generic Graph:Set Last Cursor Style", "Data"=variant} ("AlliGator Actions"), "Data"=w94) -> (w95:T8)
            n44 = Build Array(w95) -> (w96:T8[])
          }
        }
      }
      event "Pin Button": Value Change {
        n45 = event-data() -> ("NewVal"=w99:bool)  [unwired: 1 in]
        n46 = call "AlliGator Dock-Undock Subpanel Event.vi"("Dock?"=w99, "VI in"=w100) -> ("Error Out"=w98:errorcluster)  [unwired: 9 in]
      }
      event User Event {
        n47 = event-data() -> ("subpanel"=w103:string, "event"=w102:string)  [unwired: 1 in]
        n48 = case shown="\"AlliGator\"" w103 {
          tunnel: w102 -> [_ w105]
          tunnel: [_ w104] -> w101
          frame "False", Default {
          }
          frame "AlliGator" {
            n49 = case shown="\"quit\"" w105 {
              tunnel: [_ TRUE] -> w104
              frame "False", Default {
              }
              frame "quit" {
              }
            }
          }
        }
      }
      event Mouse Enter {
        n50 = event-data() -> ("CtlRef"=w108:refnum<vi>)  [unwired: 1 in]
        n51 = Unbundle By Name(w109) -> ("Event Registration Refnum"=w111:refnum<event-registration>)
        n52 = call "XY Graph Tipstrip Mouse Enter.vi"("Event Registration Refnum"=w111, "XY Graph Refnum"=w108) -> ("Event Registration Refnum"=w110:refnum<event-registration>)  [unwired: 8 in, 1 out]
        n53 = Bundle By Name(cluster=w109, "Event Registration Refnum"=w110) -> (w107:T3)
      }
      event Mouse Leave {
        n54 = event-data() -> ("CtlRef"=w113:refnum<vi>)  [unwired: 1 in]
        n55 = Unbundle By Name(w114) -> ("Event Registration Refnum"=w115:refnum<event-registration>)
        n56 = call "XY Graph Tipstrip Mouse Leave.vi"("Event Registration Refnum"=w115, "XY Graph Refnum"=w113) -> ("Event Registration Refnum"=w116:refnum<event-registration>)  [unwired: 8 in, 1 out]
        n57 = Bundle By Name(cluster=w114, "Event Registration Refnum"=w116) -> (w112:T3)
      }
      event Mouse Move {
        n58 = event-data() -> ("CtlRef"=w119:refnum<vi>, "Coords"=w118:T6)  [unwired: 1 in]
        n59 = control-ref of="Decay Graph TipStrip"() -> (w117:refnum<vi>)
        n60 = call "XY Graph Set Plot TipStrip.vi"("TipStrip Refnum"=w117, "Max Length (200)"=300, "Coords"=w118, "XY Graph Refnum"=w119) -> ()  [unwired: 5 in, 3 out]
      }
    }
    n61 = call "AlliGator Settings Storage.vi"("AlliGator Settings List"=AlliGator_Settings_List."Miscellaneous:Verbose Error Mode") -> ("Variant Data out"=w48:variant)  [unwired: 9 in, 1 out]
    n62 = call-poly "Variant to Data.vi"("Variant"=w48) -> ("Value"=w41:bool)  [unwired: 8 in]
    n63 = call "Send Message to Notebook.vi"("Error In"=w43, "Text"=w40, "Notebook Queue"=w42) -> ("Error Out"=w45:errorcluster, "Notebook Queue"=w44:refnum<queue>)  [unwired: 5 in]
    n64 = call "Light Theme Message Style.vi"() -> ()  [unwired: 1 out]
    n65 = call "AlliGator Queue Non Empty Events.vi"("Actions"=w38, "AlliGator Q"=w39) -> ()  [unwired: 9 in, 1 out]
    n66 = call "Send Error to Notebook.vi"("error in (no error)"=w45, "Verbose Error Messages (T)"=w41, "State Machine Case Error Source"="Decay Graph", "Notebook Q"=w44) -> ("Error Out"=w32:errorcluster)  [unwired: 7 in]
  }
  n67 = call "Tiny Clear Error.vi"("Error In"=w25) -> ("no Error Out"=w24:errorcluster)  [unwired: 8 in]
  n68 = Unregister For Events(event registration refnum=w26) -> (error out=w14:errorcluster)  [unwired: 1 in]
  n69 = invoke class="VI" method="FP.Close"(reference=w10, error in=w24) -> (error out=w15:errorcluster)  [unwired: 1 in, 2 out]
  n70 = Merge Errors(w15, w14) -> (w13:errorcluster)
  n71 = call "Tiny Clear Error.vi"("Error In"=w13) -> ()  [unwired: 8 in, 1 out]
